vi "Start Reader.vi"(8 "error in (no error)":errorcluster, 11 "CAN RW CANsub in":refnum<class "CAN RW CANsub.lvclass">) -> (0 "error out":errorcluster, 3 "CAN RW CANsub out":refnum<class "CAN RW CANsub.lvclass">)   [LabVIEW 2021, in "CAN RW CANsub.lvclass"]
uses:
  CAN RW CANsub.lvclass
  CAN RW CANsub.lvclass/CAN RW CANsub.ctl
  CANsub/c_client/api/CANsub_Channel/CANsub_Channel.lvclass
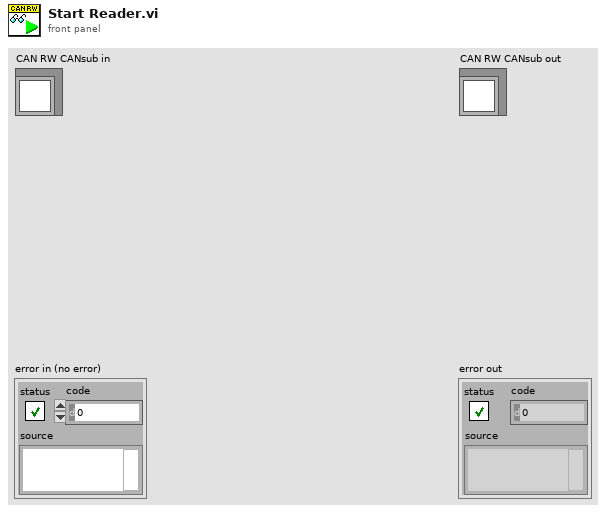
[diagram p1: front panel]
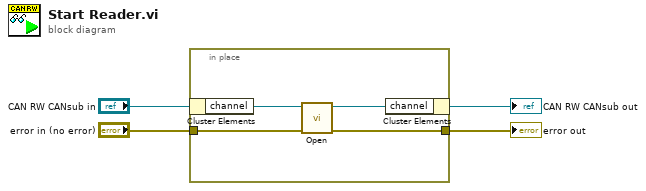
[diagram p0: block diagram]
diagram:
  n1 = in-place {
    in-place-border: "error in (no error)" -> [w7]
    in-place-border: [w5] -> w2
    n2 = in-place-cluster #1("CAN RW CANsub in") -> ("channel"=w8:refnum<class "CANsub_Channel.lvclass">)
    n3 = call-dynamic "Open.vi"("error in (no error)"=w7, "channel in"=w8) -> ("error out"=w5:errorcluster, "channel out"=w6:refnum<class "CANsub_Channel.lvclass">)  [unwired: 8 in]
    n4 = in-place-cluster #1("channel"=w6) -> (→"CAN RW CANsub out":refnum<class "CAN RW CANsub.lvclass">)
  }
  "error out" <- w2
